vi "FRC Set Systemcore Target.vi"(8 "error in (no error)":errorcluster, 9 "Team number":string, 10 "project folder":path) -> (0 "error out":errorcluster)   [LabVIEW 2023]
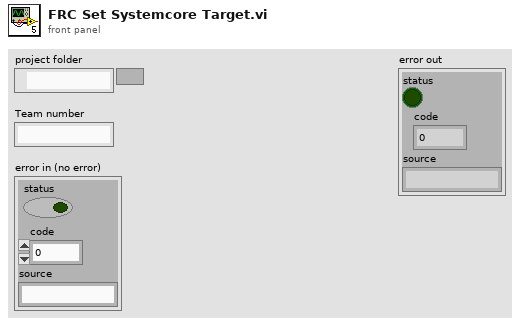
[diagram p1: front panel]
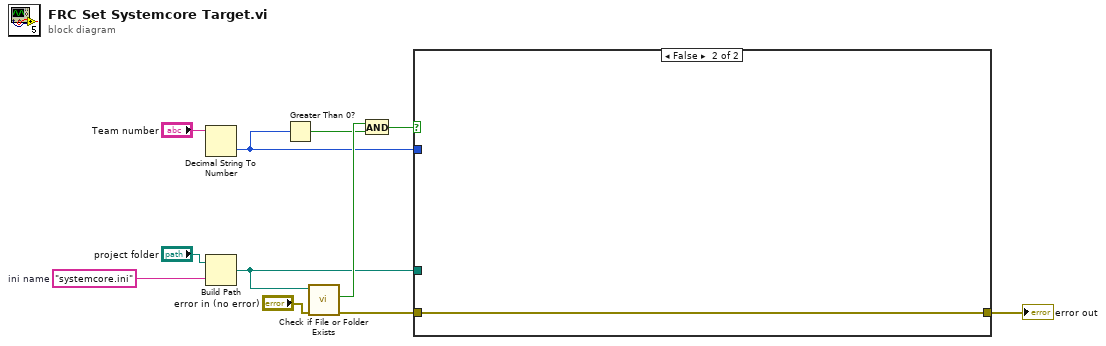
[diagram p0: block diagram]
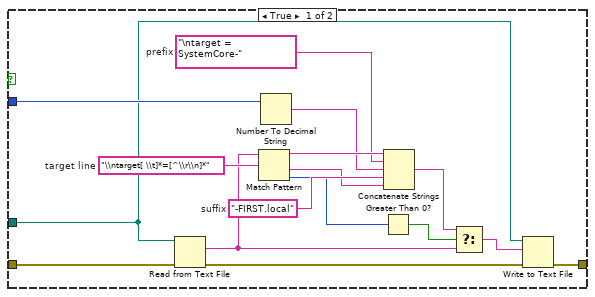
[diagram p2: hidden frame]
diagram:
  w9 = "systemcore.ini"  # ini name
  n1 = Decimal String To Number(string="Team number") -> (number=w4:i32)  [unwired: 2 in, 1 out]
  n2 = Build Path(base path="project folder", name or relative path=w9) -> (appended path=w5:path)
  n3 = Greater Than 0?(x=w4) -> (x > 0?=w6:bool)
  n4 = call <vilib>:"Check if File or Folder Exists.vi"("error in (no error)"="error in (no error)", "path"=w5) -> ("error out"=w3:errorcluster, "file or folder exists?"=w7:bool)  [unwired: 7 in, 1 out]
  n5 = And(x=w7, y=w6) -> (x .and. y?=w2:bool)
  n6 = case shown="False" w2 {
    tunnel: w5 -> [w15 _]
    tunnel: w4 -> [w27 _]
    tunnel: w3 -> [w26 w28]
    tunnel: [w12 w28] -> w1
    frame True {
      w21 = "-FIRST.local"  # suffix
      w23 = "\ntarget = SystemCore-"  # prefix
      w25 = "\\ntarget[ \\t]*=[^\\r\\n]*"  # target line
      n7 = Read from Text File(file (use dialog)=w15, error in=w26) -> (text=w16:string, error out=w13:errorcluster)  [unwired: 2 in, 2 out]
      n8 = Match Pattern(string=w16, regular expression=w25) -> (before substring=w24:string, after substring=w20:string, offset past match=w19:i32)  [unwired: 1 in, 1 out]
      n9 = Number To Decimal String(number=w27) -> (decimal integer string=w22:string)  [unwired: 1 in]
      n10 = Greater Than 0?(x=w19) -> (x > 0?=w17:bool)
      n11 = Concatenate Strings(w24, w23, w22, w21, w20) -> (w18:string)
      n12 = Select(t=w18, s=w17, f=w16) -> (s? t:f=w14:string)
      n13 = Write to Text File(file (use dialog)=w15, text=w14, error in=w13) -> (error out=w12:errorcluster)  [unwired: 1 in, 2 out]
    }
    frame False {
    }
  }
  "error out" <- w1
